vi "Format Http Request.vi"(0 "WS URI":string="ws://hostname.domain:80/resource/name", 2 "header string in":string, 3 "WebSocket Key":string="dKP/0gJzWzXMAh6SYdQ/sA==", 5 "error in":errorcluster, 9 "Relative URI Request (F)":bool) -> (14 "Secure":bool, 16 "Http Request":string, 19 "error out":errorcluster)   [LabVIEW 2021, in "LV WebSockets.lvlib"]
uses:
  LV WebSockets.lvlib
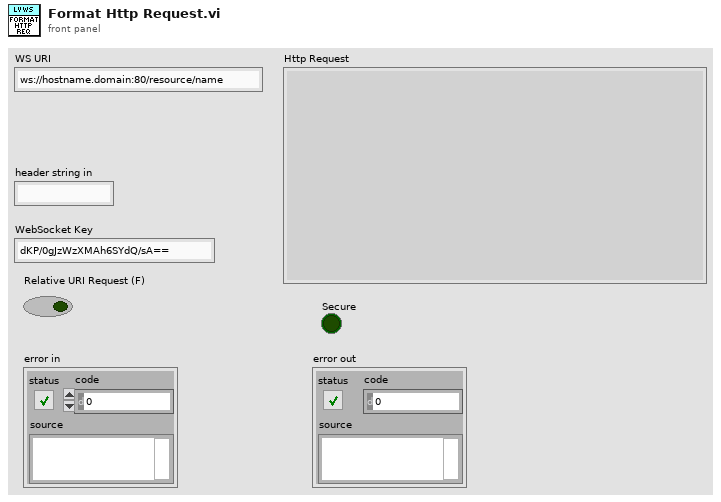
[diagram p1: front panel]
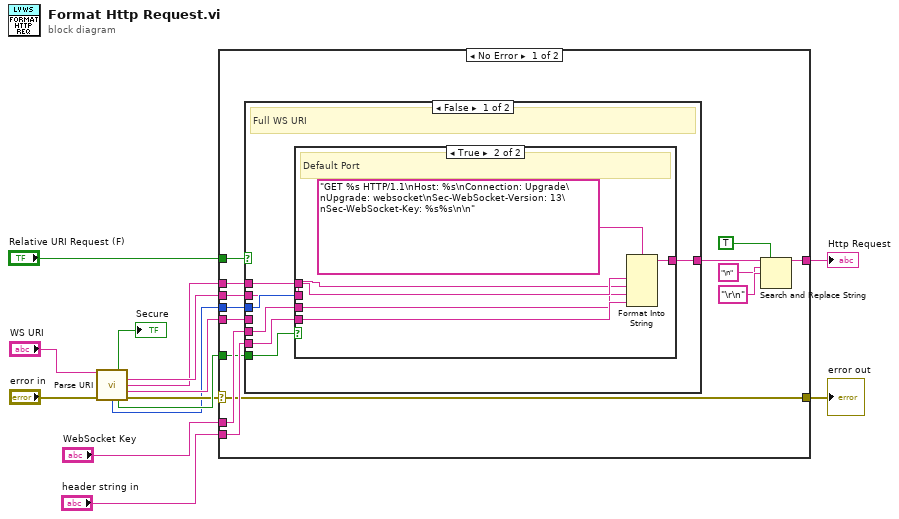
[diagram p0: block diagram]
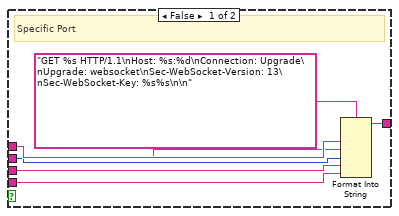
[diagram p2: hidden frame]
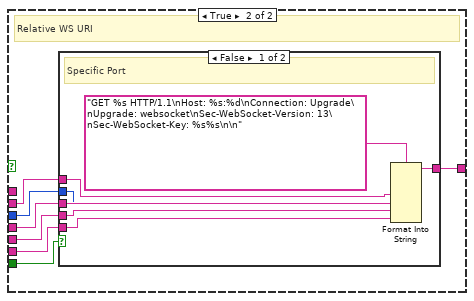
[diagram p3: hidden frame]
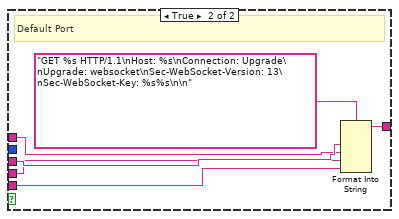
[diagram p4: hidden frame]
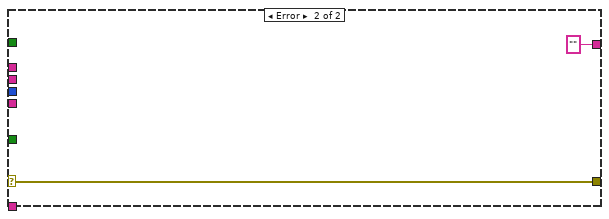
[diagram p5: hidden frame]
diagram:
  n1 = call "Parse URI.vi"("URI"="WS URI", "error in"="error in") -> ("Secure"=→"Secure":bool, "Hostname"=w9:string, "HTTP URI"=w2:string, "Resource Name"=w4:string, "Port"=w3:u16, "Default Port"=w7:bool, "error out"=w6:errorcluster)  [unwired: 6 in, 1 out]
  n2 = case shown="No Error" w6 {
    selector: w6 -> [w16 w70]
    tunnel: "header string in" -> [w28 _]
    tunnel: "WebSocket Key" -> [w25 _]
    tunnel: [w23 "" ("result string")] -> w12
    tunnel: "Relative URI Request (F)" -> [w21 _]
    tunnel: w3 -> [w20 _]
    tunnel: w2 -> [w19 _]
    tunnel: w9 -> [w18 _]
    tunnel: w7 -> [w17 _]
    tunnel: [w16 w70] -> w5
    tunnel: w4 -> [w15 _]
    frame No Error {
      n3 = case shown="False" w21 {
        tunnel: w20 -> [w35 w51]
        tunnel: w19 -> [w34 _]
        tunnel: w28 -> [w33 w55]
        tunnel: w25 -> [w32 w54]
        tunnel: [w31 w53] -> w24
        tunnel: w18 -> [w29 w52]
        tunnel: w17 -> [w30 w50]
        tunnel: w15 -> [_ w49]
        frame False {
          # "Full WS URI"
          n4 = case shown="True" w30 {
            tunnel: w35 -> [w37 _]
            tunnel: w34 -> [w42 w48]
            tunnel: w33 -> [w41 w47]
            tunnel: w32 -> [w40 w46]
            tunnel: [w38 w44] -> w31
            tunnel: w29 -> [w36 w43]
            frame False {
              # "Specific Port"
              n5 = Format Into String(format string="GET %s HTTP/1.1\nHost: %s:%d\nConnection: Upgrade\nUpgrade: websocket\nSec-WebSocket-Version: 13\nSec-WebSocket-Key: %s%s\n\n", w42, w36, w37, w40, w41) -> (resulting string=w38:string)  [unwired: 2 in, 1 out]
            }
            frame True {
              # "Default Port"
              n6 = Format Into String(format string="GET %s HTTP/1.1\nHost: %s\nConnection: Upgrade\nUpgrade: websocket\nSec-WebSocket-Version: 13\nSec-WebSocket-Key: %s%s\n\n", w48, w43, w46, w47) -> (resulting string=w44:string)  [unwired: 2 in, 1 out]
            }
          }
        }
        frame True {
          # "Relative WS URI"
          n7 = case shown="False" w50 {
            tunnel: w49 -> [w62 w68]
            tunnel: w55 -> [w61 w67]
            tunnel: w54 -> [w60 w66]
            tunnel: [w58 w64] -> w53
            tunnel: w52 -> [w57 w63]
            tunnel: w51 -> [w56 _]
            frame False {
              # "Specific Port"
              n8 = Format Into String(format string="GET %s HTTP/1.1\nHost: %s:%d\nConnection: Upgrade\nUpgrade: websocket\nSec-WebSocket-Version: 13\nSec-WebSocket-Key: %s%s\n\n", w62, w57, w56, w60, w61) -> (resulting string=w58:string)  [unwired: 2 in, 1 out]
            }
            frame True {
              # "Default Port"
              n9 = Format Into String(format string="GET %s HTTP/1.1\nHost: %s\nConnection: Upgrade\nUpgrade: websocket\nSec-WebSocket-Version: 13\nSec-WebSocket-Key: %s%s\n\n", w68, w63, w66, w67) -> (resulting string=w64:string)  [unwired: 2 in, 1 out]
            }
          }
        }
      }
      n10 = Search and Replace String(replace all?=TRUE ("replace all? (F)"), input string=w24, search string="\n", replace string="\r\n" ("replace string (\"\")")) -> (result string=w23:string)  [unwired: 4 in, 3 out]
    }
    frame Error {
    }
  }
  "Http Request" <- w12
  "error out" <- w5
